vi "CE Math - General Error Handler.vi"(5 "hierarhy level":i32=1, 6 "error before":errorcluster, 7 "error code":i32=1, 8 "message":string, 9 "error? (T)":bool=TRUE) -> (0 "error out":errorcluster, 3 "error status":bool=TRUE)   [LabVIEW 2021]
doc: "::: CalcExpress Toolkit :::\nCopyright (c) 2000-2026 Konstantin Shifershteyn. All rights reserved."
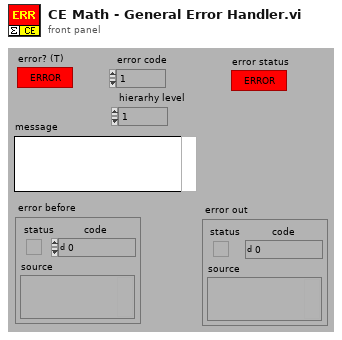
[diagram p1: front panel]
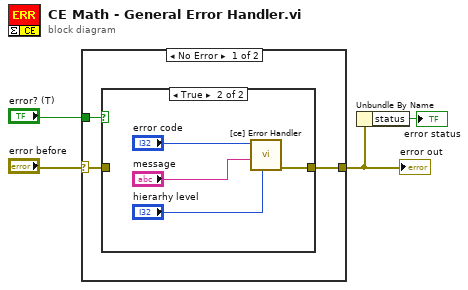
[diagram p0: block diagram]
diagram:
  n1 = case shown="No Error" "error before" {
    selector: "error before" -> [w5 w13]
    tunnel: [w7 w13] -> w2
    tunnel: "error? (T)" -> [w6 _]
    frame No Error {
      n2 = case shown="True" w6 {
        tunnel: [w8 w9] -> w7
        tunnel: w5 -> [w8 _]
        frame False {
        }
        frame True {
          n3 = call "[ce] Error Handler.vi"("nesting level"="hierarhy level", "error reason"="message", "error code"="error code") -> ("error out"=w9:errorcluster)  [unwired: 7 in, 1 out]
        }
      }
    }
    frame Error {
    }
  }
  "error out" <- w2
  n4 = Unbundle By Name(w2) -> ("status"=→"error status":bool)
